vi "set OBW X dB Value.vi"(8 "error in (no error)":errorcluster, 10 "OBW X dB (minus Value)":dbl, 11 "Keysight 9020A in":refnum<class "Keysight 9020A.lvclass">) -> (0 "error out":errorcluster, 3 "Keysight 9020A out":refnum<class "Keysight 9020A.lvclass">)   [LabVIEW 2023, in "Spectrum Analyzer.lvlib" / "Keysight 9020A.lvclass"]
uses:
  Keysight 9020A.lvclass
  Keysight 9020A.lvclass/Keysight 9020A.ctl
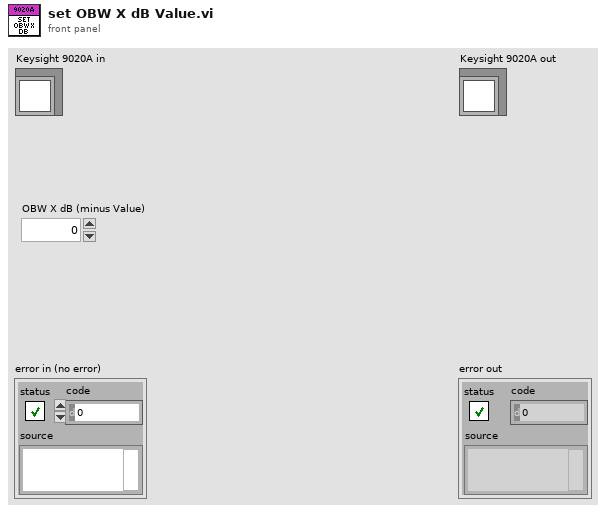
[diagram p1: front panel]
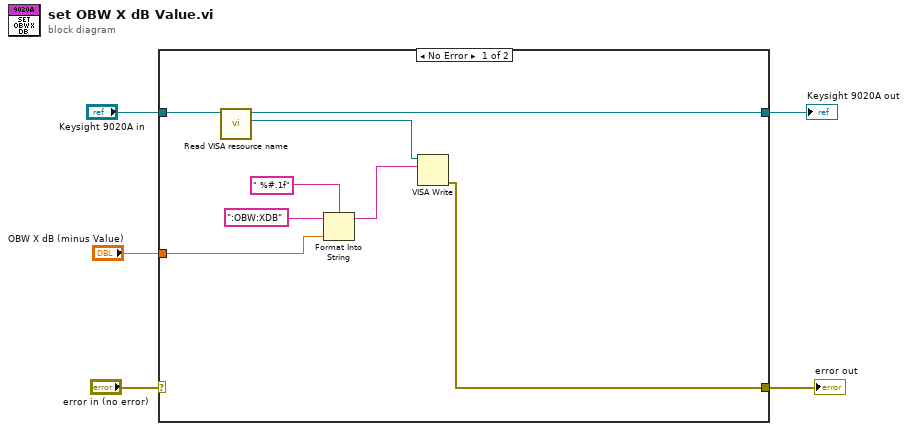
[diagram p0: block diagram]
diagram:
  n1 = case shown="No Error" "error in (no error)" {
    selector: "error in (no error)" -> [_ w14]
    tunnel: "Keysight 9020A in" -> [w13 w15]
    tunnel: [w12 w15] -> w4
    tunnel: [w8 w14] -> w2
    tunnel: "OBW X dB (minus Value)" -> [w6 _]
    frame No Error {
      n2 = call "Read VISA resource name.vi"("Keysight 9020A in"=w13) -> ("VISA resource name"=w9:refnum<visa-resource-name>, "Keysight 9020A out"=w12:refnum<class "Keysight 9020A.lvclass">)  [unwired: 8 in, 1 out]
      n3 = Format Into String(format string=" %#.1f", initial string=":OBW:XDB" ("string"), w6) -> (resulting string=w11:string)  [unwired: 1 in, 1 out]
      n4 = VISA Write(VISA resource name=w9, write buffer=w11) -> (error out=w8:errorcluster)  [unwired: 1 in, 2 out]
    }
    frame Error {
    }
  }
  "error out" <- w2
  "Keysight 9020A out" <- w4
